vi "libssh2_agent_get_identity.vi"(8 "error in (no error)":errorcluster, 10 "prev":T1, 11 "agent":T2) -> (0 "error out":errorcluster, 1 "end reached":bool, 2 "store":T1)   [LabVIEW 2017, in "libssh2.lvlib"]
doc: "Get a public key off the internal list of public keys. Call <B>libssh2_agent_list_identities</B> to request a list of public keys from the SSH agent."
uses:
  libssh2.lvlib
  Agent Refnum.ctl
  Agent Public Key Refnum.ctl
  Acquire Session.vi
  Release Session.vi
  Not An Agent.vi
  <vilib>/Utility/error.llb/Error Cluster From Error Code.vi
  Global Settings.vi
  Read Agent Refnum.vi
  Read Session Refnum.vi
  <vilib>/Utility/semaphor.llb/Acquire Semaphore.vi
  <vilib>/Utility/semaphor.llb/Release Semaphore.vi
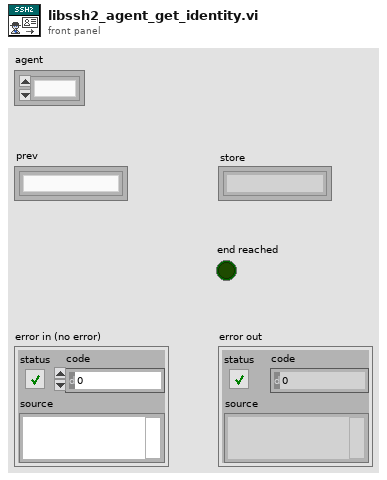
[diagram p1: front panel]
types:
  T1 = typedef "libssh2.lvlib/Agent Public Key Refnum.ctl" = refnum<k1>
  T2 = typedef "libssh2.lvlib/Agent Refnum.ctl" = refnum<k1>
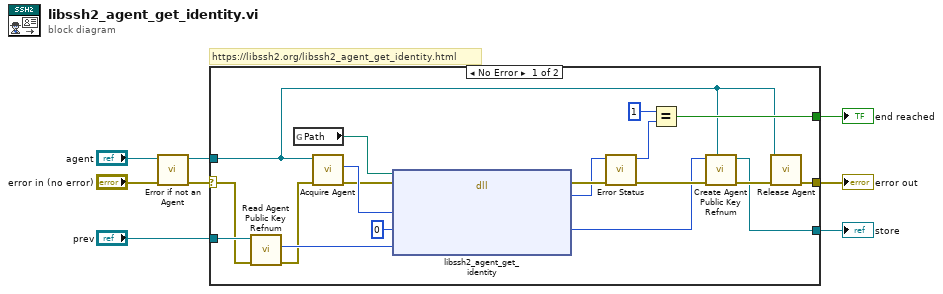
[diagram p0: block diagram]
diagram:
  # "https://libssh2.org/libssh2_agent_get_identity.html"
  n1 = call "Error if not an Agent.vi"("error in (no error)"="error in (no error)", "agent"="agent") -> ("error out"=w3:errorcluster, "agent out"=w1:T2)  [unwired: 8 in]
  n2 = case shown="No Error" w3 {
    selector: w3 -> [w13 w28]
    tunnel: w1 -> [w9 _]
    tunnel: [w10 w28] -> w8
    tunnel: [w26 _] -> w6
    tunnel: [w25 _] -> w5
    tunnel: "prev" -> [w24 _]
    frame No Error {
      n3 = call "Read Agent Public Key Refnum.vi"("error in (no error)"=w13, "agent public key"=w24) -> ("error out"=w12:errorcluster, "libssh2_agent_publickey*"=w15:u64)  [unwired: 7 in, 1 out]
      n4 = global read "Global Settings.vi" "Path"() -> (w23:path)
      n5 = call "Acquire Agent.vi"("error in (no error)"=w12, "agent"=w9) -> ("error out"=w14:errorcluster, "LIBSSH2_AGENT*"=w22:u64)  [unwired: 8 in]
      n6 = dll-call lib="?" fn="libssh2_agent_get_identity"(path in=w23, error in=w14, "agent"=w22, "store"=u64 0, "prev"=w15) -> (error out=w19:errorcluster, "return value"=w18:i32, "store"=w16:u64)  [unwired: 3 in, 1 out]
      n7 = call "Error Status.vi"("error in (no error)"=w19, "return value"=w18) -> ("error out"=w17:errorcluster, "return value out"=w20:i32)  [unwired: 8 in]
      n8 = Equal?(x=1, y=w20) -> (x = y?=w26:bool)
      n9 = call "Create Agent Public Key Refnum.vi"("agent"=w9, "error in (no error)"=w17, "libssh2_agent_publickey*"=w16) -> ("error out"=w27:errorcluster, "agent public key"=w25:T1)  [unwired: 7 in]
      n10 = call "Release Agent.vi"("error in (no error)"=w27, "agent"=w9) -> ("error out"=w10:errorcluster)  [unwired: 9 in]
    }
    frame Error {
    }
  }
  "error out" <- w8
  "end reached" <- w6
  "store" <- w5
